vi "App_Init.vi"(11 "error in":errorcluster) -> (4 "Channels":T1, 15 "error out":errorcluster)   [LabVIEW 2020, in "GH_App.lvlib"]
doc: "Start of Main: creates the key queue (UI to engine), the notifier (game state for the picture loop) and the sound queue (sound bits for the audio loop) and returns them as Channels."
uses:
  GH_App.lvlib
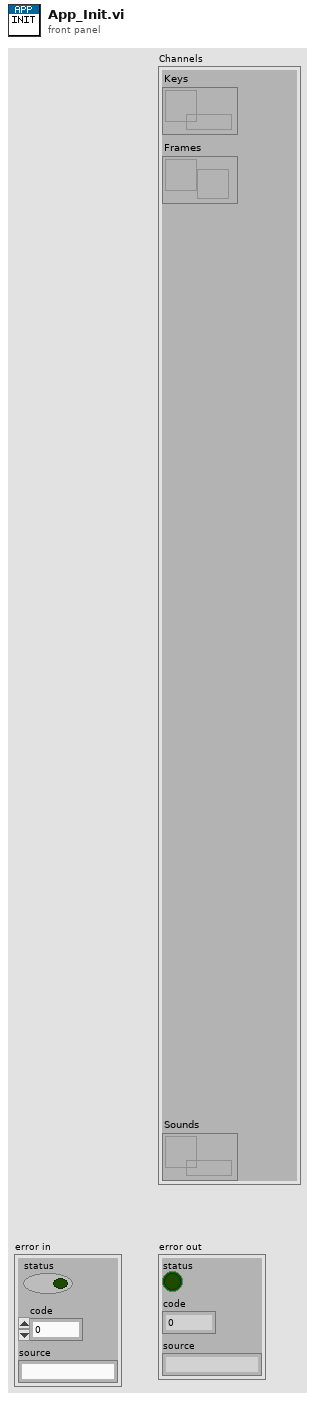
[diagram p1: front panel]
types:
  T1 = cluster{"Keys":refnum<queue>, "Frames":refnum<notifier>, "Sounds":refnum<queue>}
  T2 = cluster{"Tick":u32, "Phase":i32, "PhaseTicks":i32, "Level":i32, "Room":i32, "X10":i32, "Y10":i32, "VY10":i32, "Mode":i32, "Facing":i32, "Run":i32, "Vert":i32, "StandY":i32, "EntryX10":i32, "EntryY10":i32, "EntryMode":i32, "Lives":i32, "Score":i32, "NextLife":i32, "KeyR":i32, "KeyB":i32, "KeyY":i32, "Torch":bool, "FloorPhase":i32, "Dead":bool, "LevelStart":bool, "Quit":bool, "Sound":i32, "Seed":u32, "DemoStep":i32, "Tiles":u8[][], "World":cluster{"ID":string, "Depth":i32, "Column":i32, "Tiles":u8[][]}[], "Enemies":cluster{"Kind":i32, "X10":i32, "Y10":i32, "Dir":i32, "Mode":i32}[], "Highscores":cluster{"Score":i32, "Name":string}[], "Name":i32[], "Cursor":i32}
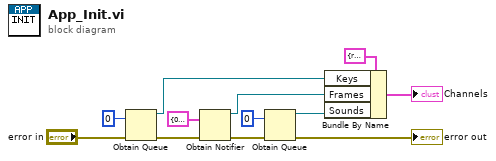
[diagram p0: block diagram]
diagram:
  n1 = Obtain Queue(element data type=u16 0 ("Key type"), error in (no error)="error in") -> (queue out=w3:refnum<queue>, error out=w4:errorcluster)  [unwired: 3 in, 1 out]
  n2 = Obtain Notifier(notification data type=T2 {"Tick"=0, "Phase"=0, "PhaseTicks"=0, "Level"=1, "Room"=0, "X10"=0, "Y10"=0, "VY10"=0, "Mode"=0, "Facing"=0, "Run"=0, "Vert"=0, "StandY"=0, "EntryX10"=0, "EntryY10"=0, "EntryMode"=0, "Lives"=4, "Score"=0, "NextLife"=10000, "KeyR"=0, "KeyB"=0, "KeyY"=0, "Torch"=FALSE, "FloorPhase"=0, "Dead"=FALSE, "LevelStart"=FALSE, "Quit"=FALSE, "Sound"=0, "Seed"=12345, "DemoStep"=0, "Tiles"=[], "World"=[], "Enemies"=[], "Highscores"=[], "Name"=[0, 0, 0], "Cursor"=0} ("State type"), error in (no error)=w4) -> (notifier out=w6:refnum<notifier>, error out=w7:errorcluster)  [unwired: 2 in, 1 out]
  n3 = Obtain Queue(element data type=0 ("Sound type"), error in (no error)=w7) -> (queue out=w9:refnum<queue>, error out=→"error out":errorcluster)  [unwired: 3 in, 1 out]
  n4 = Bundle By Name(cluster=T1 {"Keys"=refnum, "Frames"=refnum, "Sounds"=refnum}, "Keys"=w3, "Frames"=w6, "Sounds"=w9) -> (→"Channels":T1)
